vi "Unregister All.vi"(8 "error in (no error)":errorcluster) -> (0 "error out":errorcluster, 3 "loggers":refnum<class "Logger.lvclass">[](array[class]))   [LabVIEW 2018, in "GLog.lvlib" / "Registry.lvlib"]
uses:
  Registry.lvlib
  api/logger_class/Logger.lvclass
  Registry Actions.ctl
  Registry Global.vi
panel:
  # "Connector Pane"
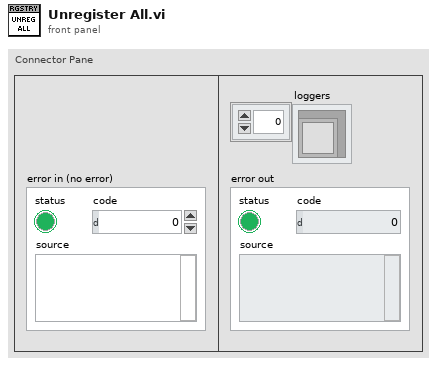
[diagram p1: front panel]
types:
  T1 = typedef "GLog.lvlib/Registry.lvlib/Registry Actions.ctl" = enum16{"Register", "Log", "Enable", "Enable All", "Disable", "Disable All", "Get Enable State", "Get Minimum Log Level", "Set Minimum Log Level", "Set All Minimum Log Level", "Get Logger Info", "Get All Logger Info", "List", "Unregister", "Unregister All", "Shutdown"}
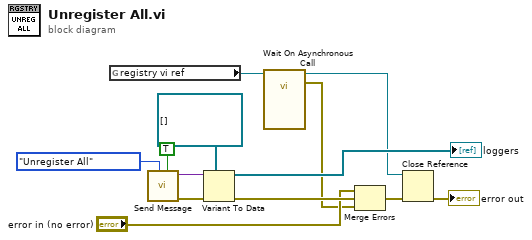
[diagram p0: block diagram]
diagram:
  n1 = global read "Registry Global.vi" "registry vi ref"() -> (w4:refnum<vi>)
  n2 = call "Send Message.vi"("return data? (F)"=TRUE, "action"=Registry_Actions."Unregister All") -> ("error out"=w8:errorcluster, "Variant"=w12:variant)  [unwired: 8 in]
  n3 = Variant To Data(error in=w8, type=refnum<class "Logger.lvclass">[] [] ("Array"), Variant=w12) -> (data=→"loggers":refnum<class "Logger.lvclass">[], error out=w7:errorcluster)
  n4 = call-by-ref "Wait On Asynchronous Call"(reference=w4) -> (reference out=w1:refnum<vi>, error out=w3:errorcluster)  [unwired: 13 in]
  n5 = Merge Errors("error in (no error)", w7, w3) -> (w6:errorcluster)
  n6 = Close Reference(reference=w1, error in (no error)=w6) -> (error out=→"error out":errorcluster)
